vi "DF002 - Constant string creator.vi"   [LabVIEW 2015]
uses:
  <vilib>/Utility/file.llb/Read Delimited Spreadsheet (string).vi
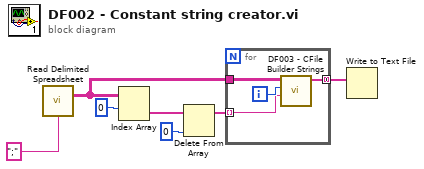
[diagram p0: block diagram]
diagram:
  n1 = call-poly <vilib>:"Read Delimited Spreadsheet.vi"("delimiter (\\t)"=";" ("delimiter (\\t)")) -> ("all rows"=w7:string[][])  [unwired: 9 in, 5 out]
  n2 = Index Array(array=w7, index (row)=0 ("index")) -> (element=w3:string[])  [unwired: 1 in]
  n3 = Delete From Array(array=w3, index=0) -> (array with subset deleted=w6:string[])  [unwired: 1 in, 1 out]
  n4 = for {
    tunnel: w7 -> [w11]
    tunnel: w6 -> [w9] mode=indexing
    tunnel: [w8] -> w1 mode=concatenating
    i -> [w10]
    n5 = call "DF003 - CFile Builder Strings.vi"("Language Prefix"=w9, "Value Row Index"=w10, "Input Table (String Array)"=w11) -> ("Generated Constant Strings"=w8:string[])  [unwired: 8 in]
  }
  n6 = Write to Text File(text=w1) -> ()  [unwired: 3 in, 3 out]
